vi "Create Message Data Clusters.vi"(8 "error in (no error)":errorcluster, 9 "generate serialization helpers":bool, 10 "message parameters":T1[](array[typedef]), 11 "library in":refnum<vi>) -> (0 "error out":errorcluster, 3 "library out":refnum<vi>)   [LabVIEW 2019, in "gRPC Template Creation Utility.lvlib"]
uses:
  gRPC Template Creation Utility.lvlib
  TypeDefs/Message Metadata (Scripting).ctl
  TypeDefs/Message Element Metadata (Scripting).ctl
  TypeDefs/Message Element Type.ctl
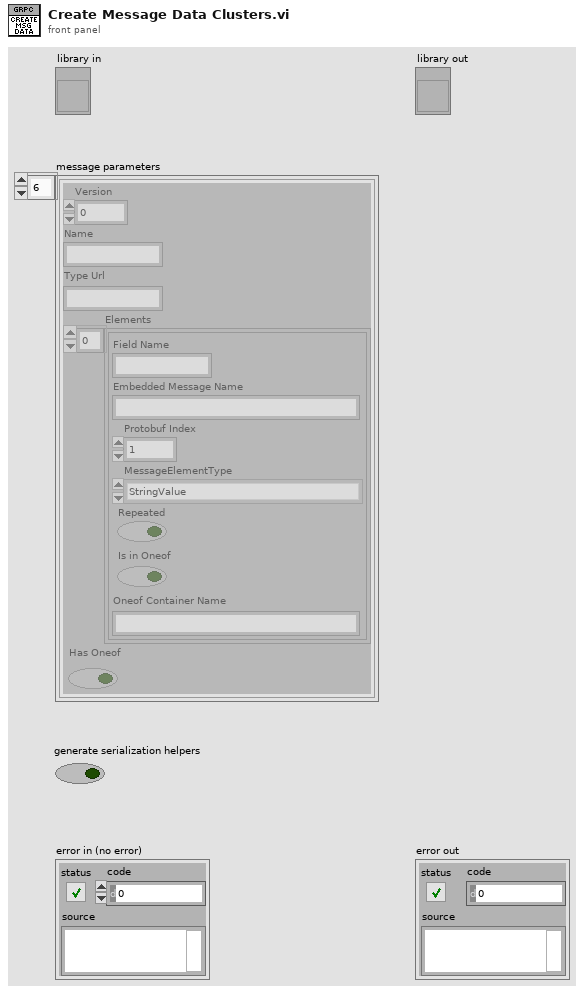
[diagram p1: front panel]
types:
  T1 = typedef "gRPC Template Creation Utility.lvlib/Message Metadata (Scripting).ctl" = cluster{"Version":i32, "Name":string, "Type Url":string, "Elements":T2[], "Has Oneof":bool}
  T2 = typedef "gRPC Template Creation Utility.lvlib/Message Element Metadata (Scripting).ctl" = cluster{"Field Name":string, "Embedded Message Name":string, "Protobuf Index":i32, "MessageElementType":T3, "Repeated":bool, "Is in Oneof":bool, "Oneof Container Name":string}
  T3 = typedef "gRPC Template Creation Utility.lvlib/Message Element Type.ctl" = enum32{"Int32Value", "FloatValue", "DoubleValue", "BoolValue", "StringValue", "MessageValue", "Int64Value", "UInt32Value", "UInt64Value", "EnumValue", "Bytes", "Fixed64", "Fixed32", "SFixed64", "SFixed32", "SInt64", "SInt32"}
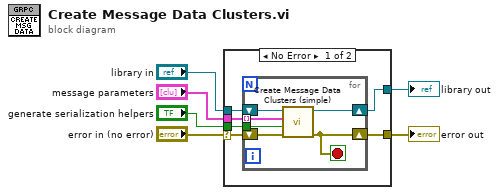
[diagram p0: block diagram]
diagram:
  n1 = case shown="No Error" "error in (no error)" {
    selector: "error in (no error)" -> [w8 w19]
    tunnel: "message parameters" -> [w12 _]
    tunnel: [w10 w20] -> w5
    tunnel: [w11 w19] -> w4
    tunnel: "library in" -> [w9 w20]
    tunnel: "generate serialization helpers" -> [w7 _]
    frame No Error {
      n2 = for {
        shift-right: [w16] -> w10
        shift-left: w9 -> [w18]
        shift-right: [w15] -> w11
        shift-left: w8 -> [w17]
        tunnel: w12 -> [w14] mode=indexing
        tunnel: w7 -> [w13]
        stop <- w15 stop-if-true
        n3 = call "Create Message Data Clusters (simple).vi"("error in (no error)"=w17, "generate converters"=w13, "message metadata"=w14, "library in"=w18) -> ("error out"=w15:errorcluster, "library out"=w16:refnum<vi>)  [unwired: 6 in]
      }
    }
    frame Error {
    }
  }
  "library out" <- w5
  "error out" <- w4
